vi "SMTP Email Open Session.vi"(4 "error in (no error)":errorcluster caption="entrée d'erreur (pas d'erreur)", 5 "timeout ms (60000)":i32=60000 caption="timeout en ms (60000)", 7 "mail server":string caption="serveur mail") -> (0 "error out":errorcluster caption="sortie d'erreur", 3 "smtp session out":T1 caption="session smtp en sortie")   [LabVIEW 2022 SP3, in "Copie de NI_SMTPEmail.lvlib"]
doc: "Ouvre une connexion TCP sur le serveur SMTP spécifié comme Mailserver et envoie une commande HELO. Le VI renvoie une \"session SMTP en sortie\" et les résultats d'interprétation de l'erreur dans le cluster de sortie d'erreur."
uses:
  Copie de NI_SMTPEmail.lvlib
  SMTP Email Session.ctl
panel:
  in  "smtp session":T1 caption="session smtp"
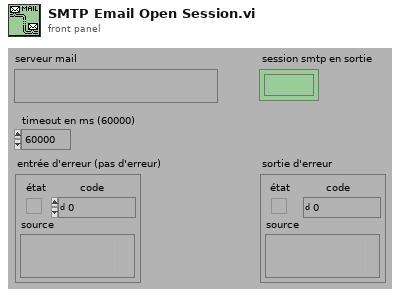
[diagram p1: front panel]
types:
  T1 = typedef "Copie de NI_SMTPEmail.lvlib/SMTP Email Session.ctl" = refnum<k1>
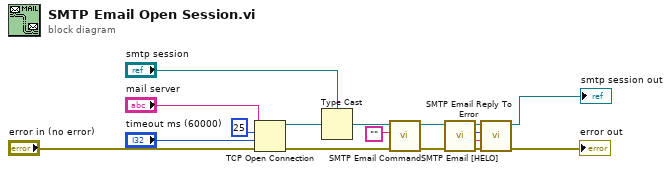
[diagram p0: block diagram]
diagram:
  n1 = TCP Open Connection(address="mail server", remote port or service name=u16 25 ("remote port"), timeout ms (60000)="timeout ms (60000)", error in (no error)="error in (no error)") -> (connection ID=w11:refnum<k5>, error out=w12:errorcluster)  [unwired: 1 in]
  n2 = Type Cast(type="smtp session", x=w11) -> (*(type *) &x=w14:T1)
  n3 = call "SMTP Email Command.vi"("error in (no error)"=w12, "command"="", "smtp session"=w14) -> ("error out"=w13:errorcluster, "smtp session out"=w9:T1)  [unwired: 1 in, 2 out]
  n4 = call "SMTP Email [HELO].vi"("error in (no error)"=w13, "smtp session"=w9) -> ("error out"=w10:errorcluster, "reply"=w8:string, "reply code"=w7:i32, "smtp session out"=w6:T1)  [unwired: 2 in]
  n5 = call "SMTP Email Reply To Error.vi"("error in (no error)"=w10, "reply string in"=w8, "reply code in"=w7, "smtp session"=w6) -> ("error out"=→"error out":errorcluster, "smtp session out"=→"smtp session out":T1)  [unwired: 2 out]
